vi "UE_Within_Tolerance.vi"(3 "tolerance":dbl, 4 "target":dbl, 5 "actual":dbl) -> (2 "within_tolerance":bool)   [LabVIEW 2026]
doc: "INTENT: Check actual within target plus or minus configured nonnegative tolerance. INPUTS: actual (double), target (double), tolerance (double). OUTPUTS: within_tolerance (bool). DESIGN CONSTRAINT: Caller checks tolerance>=0 and feedback freshness. REQUIREMENTS: SRS-F-005. No physical hardware side effects. Acceptance requires native LabVIEW compilation and behavioral testing."
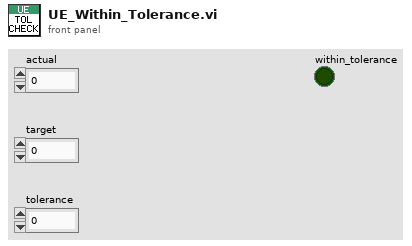
[diagram p1: front panel]
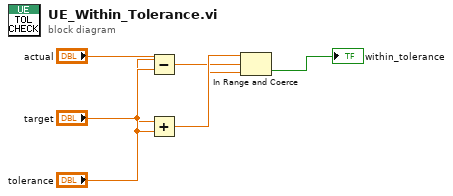
[diagram p0: block diagram]
diagram:
  n1 = Subtract(x="target", y="tolerance") -> (x-y=w4:dbl)
  n2 = Add(x="target", y="tolerance") -> (x+y=w5:dbl)
  n3 = In Range and Coerce(upper limit=w5, x="actual", lower limit=w4) -> (In Range?=→"within_tolerance":bool)  [unwired: 1 out]
